vi "Global_Stop.vi"() -> ()   [LabVIEW 2024]
panel:
  in  "stop":bool
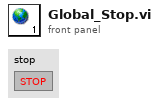
[diagram p1: front panel]
diagram:
